vi "Create Execution Unit.vi"(8 "error in":errorcluster, 10 "Item Ref":T2=18446744073709551615 format="%.0x", 11 "Execution Unit Factory Implementation in":refnum<class "Execution Unit Factory.lvclass">) -> (0 "error out":errorcluster, 1 "Asynchronous Execution Units":cluster{"Grouped Execution Units":T1[]}[](array[cluster]) {"Grouped Execution Units"."ReadWrite Channels" format="%.0x"; "Grouped Execution Units"."Outgoing Channels" format="%.0x"; "Grouped Execution Units"."Incoming Channels" format="%.0x"}, 2 "Inline Execution Units":T1[](array[typedef]) {"ReadWrite Channels" format="%.0x"; "Outgoing Channels" format="%.0x"; "Incoming Channels" format="%.0x"}, 3 "Execution Unit Factory Implementation out":refnum<class "Execution Unit Factory.lvclass">)   [LabVIEW 2020, in "AIM ARINC 429 Engine.lvlib" / "Implementation.lvlib" / "Execution Unit Factory.lvclass"]
uses:
  Execution Unit Factory.lvclass
  <vilib>/NI VeriStand/Custom Device API/Custom Device Item Ref.ctl
  Interfaces/Controls/Execution Unit Information.ctl
  Interfaces/Execution Unit/Execution Unit.lvclass
  Execution Unit/Execution Unit.lvclass
  C:/Users/nitest/Desktop/Git 2020/niveristand-aim-arinc429-custom-device/Source/Custom Device Support/Engine/Interfaces/Execution Unit/Execution Unit.lvclass
  Rx Execution Unit/Rx Execution Unit.lvclass
  Logging Execution Unit/Logging Execution Unit.lvclass
  Tx Acyclic Labels Execution Unit/Tx Acyclic Labels Execution Unit.lvclass
  C:/Users/nitest/Desktop/Git 2020/niveristand-aim-arinc429-custom-device/Source/Custom Device Support/Engine/Implementation/Execution Unit/Execution Unit.lvclass
  Tx Scheduled Labels Execution Unit/Tx Scheduled Labels Execution Unit.lvclass
  <vilib>/NI VeriStand/Custom Device API/Custom Device API.lvlib
  Interfaces/Interfaces.lvlib
  System Explorer/Implementation/Implementation.lvlib
  Scripting/AIM/AIM ARINC 429 Scripting.lvlib
  C:/Users/nitest/Desktop/Git 2020/niveristand-aim-arinc429-custom-device/Source/Custom Device Support/Engine/Implementation/Logging Execution Unit/Logging Execution Unit.lvclass
  C:/Users/nitest/Desktop/Git 2020/niveristand-aim-arinc429-custom-device/Source/Custom Device Support/Engine/Implementation/Tx Acyclic Labels Execution Unit/Tx Acyclic Labels Execution Unit.lvclass
  C:/Users/nitest/Desktop/Git 2020/niveristand-aim-arinc429-custom-device/Source/Custom Device Support/Engine/Implementation/Tx Scheduled Labels Execution Unit/Tx Scheduled Labels Execution Unit.lvclass
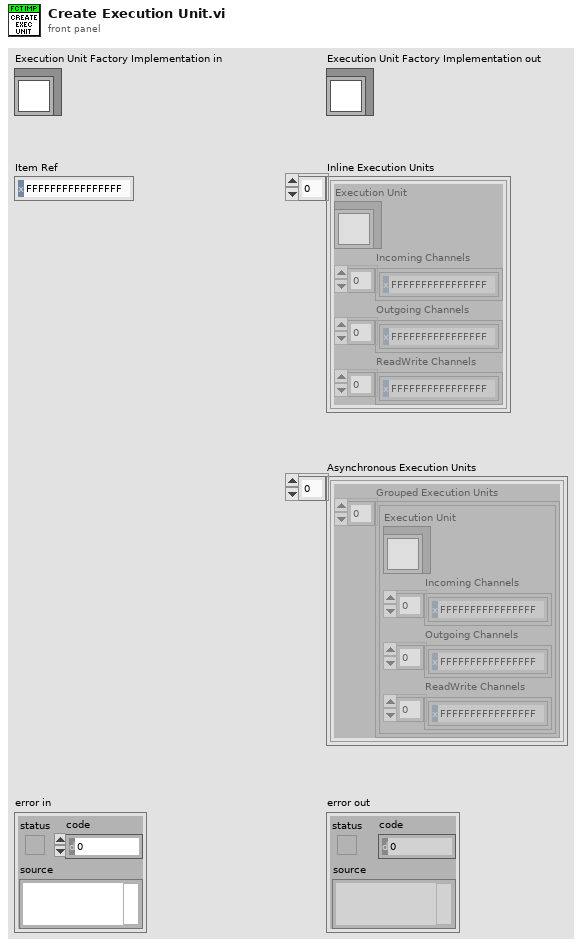
[diagram p1: front panel]
types:
  T1 = typedef "AIM ARINC 429 Engine.lvlib/Interfaces.lvlib/Execution Unit Information.ctl" = cluster{"Execution Unit":refnum<class "Execution Unit.lvclass">, "Incoming Channels":T2[], "Outgoing Channels":T2[], "ReadWrite Channels":T2[]}
  T2 = typedef "Custom Device API.lvlib/Custom Device Item Ref.ctl" = u64
  T3 = typedef "RT Hardware Channel Settings.ctl" = cluster{"channel #":u16, "channel handle":u64, "labels settings for RT":T4[], "speed":T11}
  T4 = typedef "RT Label Settings.ctl" = cluster{"Name":string, "xmlName":string, "label":T5, "transfer period":u32, "SDI_Enabled":bool, "SDI":u8, "parameter driver data":T6, "transfer type":T9, "has timestamp?":bool, "Label Disable/Trigger Channel Reference":T2, "Message Handle":u64, "Initialized?":bool, "Word Initial Raw Value":u32, "Label Timestamp Channel Data Reference":T10, "disabled":bool}
  T5 = typedef "Label.ctl" = u8
  T6 = typedef "RT Parameters.ctl" = cluster{"parameter definitions":T7[], "Tx parameter refs":T2[]}
  T7 = typedef "Parameter Definition.ctl" = cluster{"start index":i32, "size":i32, "encoding":T8, "signed":bool, "scale multiplier":dbl, "scale offset":dbl, "default value":dbl}
  T8 = typedef "Encoding and Decoding.lvlib/Encoding.ctl" = enum16{"BNR", "BCD", "Discrete"}
  T9 = typedef "Transfer Type.ctl" = enum16{"Scheduled", "Acyclic", "Block", "Strobe"}
  T10 = typedef "Custom Device API.lvlib/Data Reference.ctl" = i32
  T11 = typedef "Transfer Speed.ctl" = enum16{"LO (12.5 kb/s)", "HI (100 kb/s)"}
  T12 = cluster{"transfer type":T9, "Name":string, "hardware channel data":T3[], "Outgoing Channels":T2[], "ReadWrite Channels":T2[]}[]
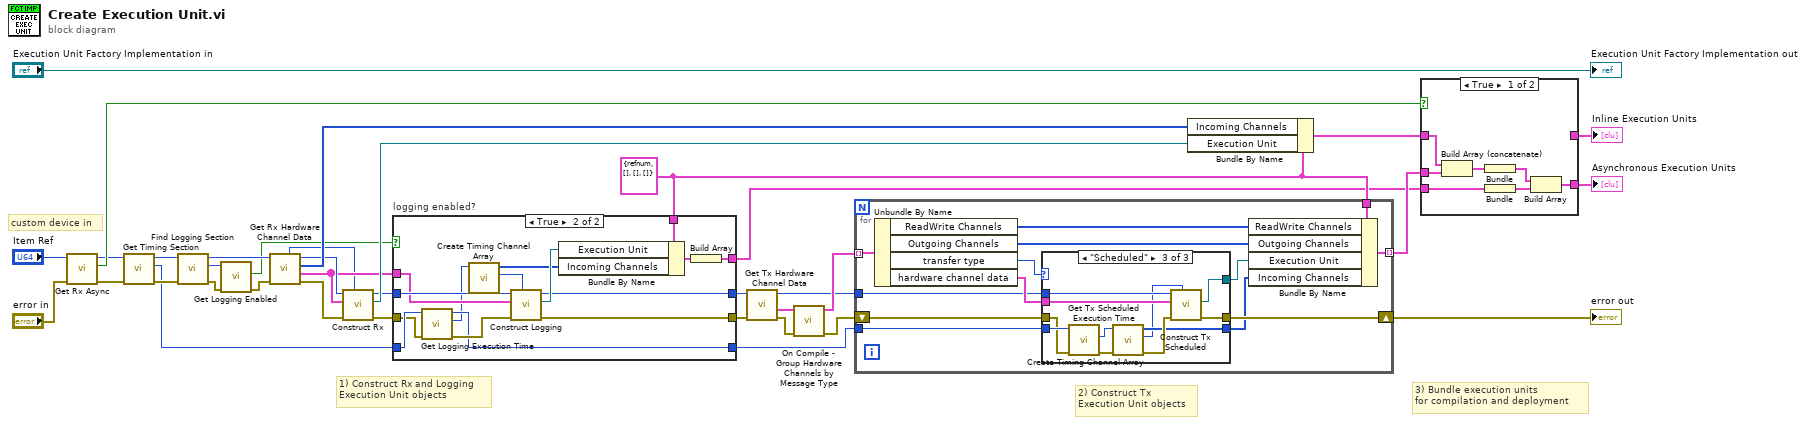
[diagram p0: block diagram]
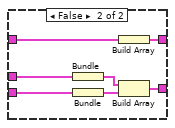
[diagram p2: hidden frame]
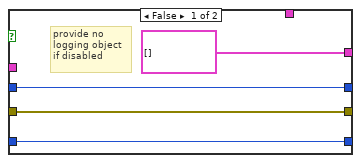
[diagram p3: hidden frame]
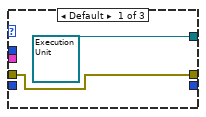
[diagram p4: hidden frame]
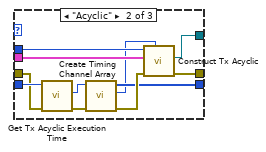
[diagram p5: hidden frame]
diagram:
  w21 = T1 {"Execution Unit"=refnum, "Incoming Channels"=[], "Outgoing Channels"=[], "ReadWrite Channels"=[]} ("Execution Unit Information")
  # "2) Construct Tx\nExecution Unit objects"
  # "custom device in"
  # "3) Bundle execution units\nfor compilation and deployment"
  # "1) Construct Rx and Logging\nExecution Unit objects"
  n1 = call "Get Rx Async.vi"("error in"="error in", "custom device ref"="Item Ref") -> ("error out"=w5:errorcluster, "rx async?"=w13:bool, "custom device ref out"=w6:T2)  [unwired: 7 in]
  n2 = call "Get Timing Section.vi"("error in"=w5, "custom device ref"=w6) -> ("error out"=w8:errorcluster, "timing"=w4:T2, "custom device ref out"=w7:T2)  [unwired: 6 in, 1 out]
  n3 = call "Find Logging Section.vi"("error in"=w8, "custom device ref"=w7) -> ("error out"=w19:errorcluster, "logging"=w18:T2, "custom device ref out"=w16:T2)  [unwired: 7 in]
  n4 = call "Get Logging Enabled.vi"("error in"=w19, "logging ref"=w18) -> ("error out"=w17:errorcluster, "logging enabled"=w15:bool)  [unwired: 7 in, 1 out]
  n5 = call "Get Rx Hardware Channel Data.vi"("error in"=w17, "custom device ref in"=w16) -> ("error out"=w34:errorcluster, "Rx hardware channel data"=w24:T3[], "incoming channels"=w35:T2[], "custom device ref out"=w28:T2, "timing channel offset"=w9:i64)  [unwired: 5 in]
  n6 = call "Construct Rx.vi"("timing channel offset (-1)"=w9, "error in"=w34, "Rx hardware channels in"=w24, "custom device ref in"=w28) -> ("error out"=w25:errorcluster, "Rx Execution Unit out"=w29:refnum<class "Rx Execution Unit.lvclass">, "custom device ref out"=w26:T2)  [unwired: 5 in]
  n7 = case "logging enabled?" shown="True" w15 {
    tunnel: w26 -> [w40 w56]
    tunnel: w25 -> [w39 w48]
    tunnel: w24 -> [_ w50]
    tunnel: [w40 w54] -> w23
    tunnel: [w39 w44] -> w22
    tunnel: w21 -> [_ w52]
    tunnel: [T1[] [] w51] -> w20
    tunnel: w4 -> [w38 w49]
    tunnel: [w38 w43] -> w3
    frame False {
      # "provide no\nlogging object\nif disabled"
    }
    frame True {
      n8 = call "Get Logging Execution Time.vi"("error in"=w48, "timing ref"=w49) -> ("error out"=w47:errorcluster, "logging execution time ref"=w42:T2, "timing ref out"=w43:T2)  [unwired: 7 in]
      n9 = call "Create Timing Channel Array.vi"("timing channel ref"=w42) -> ("channel offset"=w46:i64, "timing channel ref array"=w45:T2[])  [unwired: 9 in]
      n10 = call "Construct Logging.vi"("timing channel offset (-1)"=w46, "error in"=w47, "Logging hardware channels in"=w50, "custom device ref in"=w56) -> ("error out"=w44:errorcluster, "Logging Execution Unit out"=w55:refnum<class "Logging Execution Unit.lvclass">, "custom device ref out"=w54:T2)  [unwired: 5 in]
      n11 = Bundle By Name(cluster=w52, "Execution Unit"=w55, "Incoming Channels"=w45) -> (w53:T1)
      n12 = Build Array(w53) -> (w51:T1[])
    }
  }
  n13 = call "Get Tx Hardware Channel Data.vi"("error in"=w22, "custom device ref in"=w23) -> ("error out"=w33:errorcluster, "Tx hardware channel data"=w32:T3[], "custom device ref out"=w27:T2)  [unwired: 7 in]
  n14 = call "On Compile - Group Hardware Channels by Message Type.vi"("error in"=w33, "hardware channel data"=w32) -> ("error out"=w30:errorcluster, "hardware channel data by transfer type"=w31:T12)  [unwired: 8 in]
  n15 = for {
    tunnel: w21 -> [w68]
    tunnel: [w69] -> w36 mode=indexing
    tunnel: w31 -> [w67] mode=indexing
    shift-right: [w61] -> w2
    shift-left: w30 -> [w59]
    tunnel: w27 -> [w60]
    tunnel: w3 -> [w57]
    n16 = Unbundle By Name(w67) -> ("ReadWrite Channels"=w66:T2[], "Outgoing Channels"=w65:T2[], "transfer type"=w64:T9, "hardware channel data"=w63:T3[])
    n17 = case shown="\"Scheduled\"" w64 {
      tunnel: w63 -> [_ w81 w91]
      tunnel: [refnum<class "Execution Unit.lvclass"> refnum ("Communication Bus Template Interfaces:Implementation.lvlib:Execution Unit.lvclass") w80 w90] -> w62
      tunnel: w59 -> [w70 w77 w87]
      tunnel: [w70 w75 w85] -> w61
      tunnel: w60 -> [_ w79 w89]
      tunnel: w57 -> [_ w78 w88]
      tunnel: [_ w73 w83] -> w58
      frame Default {
      }
      frame "Acyclic" {
        n18 = call "Get Tx Acyclic Execution Time.vi"("error in"=w77, "timing ref"=w78) -> ("error out"=w76:errorcluster, "async tx execution time ref"=w74:T2)  [unwired: 7 in, 1 out]
        n19 = call "Create Timing Channel Array.vi"("timing channel ref"=w74) -> ("channel offset"=w72:i64, "timing channel ref array"=w73:T2[])  [unwired: 9 in]
        n20 = call "Construct Tx Acyclic.vi"("timing channel offset (-1)"=w72, "error in"=w76, "Tx Acyclic hardware channels in"=w81, "custom device ref in"=w79) -> ("error out"=w75:errorcluster, "Tx Acyclic Execution Unit out"=w80:refnum<class "Tx Acyclic Labels Execution Unit.lvclass">)  [unwired: 5 in, 1 out]
      }
      frame "Scheduled" {
        n21 = call "Get Tx Scheduled Execution Time.vi"("error in"=w87, "timing ref"=w88) -> ("error out"=w86:errorcluster, "sched tx execution time ref"=w84:T2)  [unwired: 7 in, 1 out]
        n22 = call "Create Timing Channel Array.vi"("timing channel ref"=w84) -> ("channel offset"=w82:i64, "timing channel ref array"=w83:T2[])  [unwired: 9 in]
        n23 = call "Construct Tx Scheduled.vi"("timing channel offset (-1)"=w82, "error in"=w86, "Tx Scheduled hardware channels in"=w91, "custom device ref in"=w89) -> ("error out"=w85:errorcluster, "Tx Scheduled Execution Unit out"=w90:refnum<class "Tx Scheduled Labels Execution Unit.lvclass">)  [unwired: 5 in, 1 out]
      }
    }
    n24 = Bundle By Name(cluster=w68, "ReadWrite Channels"=w66, "Outgoing Channels"=w65, "Execution Unit"=w62, "Incoming Channels"=w58) -> (w69:T1)
  }
  "error out" <- w2
  n25 = Bundle By Name(cluster=w21, "Incoming Channels"=w35, "Execution Unit"=w29) -> (w10:T1)
  n26 = case shown="True" w13 {
    tunnel: w36 -> [w98 w101]
    tunnel: [w94 w104] -> w12
    tunnel: w20 -> [w93 w103]
    tunnel: w10 -> [w97 w100]
    tunnel: [_ w99] -> w11
    frame True {
      n27 = Build Array (concatenate)(w97, w98) -> (w95:T1[])
      n28 = Bundle(w95) -> (w96:cluster{T1[]})  [unwired: 1 in]
      n29 = Bundle(w93) -> (w92:cluster{T1[]})  [unwired: 1 in]
      n30 = Build Array(w96, w92) -> (w94:cluster{T1[]}[])
    }
    frame False {
      n31 = Bundle(w101) -> (w105:cluster{T1[]})  [unwired: 1 in]
      n32 = Bundle(w103) -> (w102:cluster{T1[]})  [unwired: 1 in]
      n33 = Build Array(w100) -> (w99:T1[])
      n34 = Build Array(w105, w102) -> (w104:cluster{T1[]}[])
    }
  }
  "Asynchronous Execution Units" <- w12
  "Inline Execution Units" <- w11
  "Execution Unit Factory Implementation out" <- "Execution Unit Factory Implementation in"
